vi "Test Window Frame Encode.vi"   [LabVIEW 2020]
doc: "Caraya unit test of RemoteVI Window Frame Encode.vi against tests/vectors (frame.json windowFrames), generated by tests/caraya/build.py - do not edit. One Assert Equal per vector, labelled with the vector's name; expected and actual are rendered as text by support/RemoteVI Check Window Frame Encode.vi (bytes as lowercase hex), so a failure shows both in the vector's own notation."
uses:
  <vilib>/addons/_JKI Toolkits/Caraya/classes/Test/Test.lvclass
  <vilib>/addons/_JKI Toolkits/Caraya/classes/Assert/Assert.lvclass
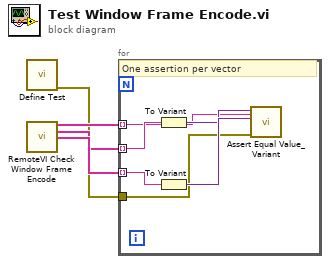
[diagram p0: block diagram]
diagram:
  n1 = call <vilib>:"Define Test.vi"() -> ("error out"=w1:errorcluster)  [unwired: 10 in, 1 out]
  n2 = call "RemoteVI Check Window Frame Encode.vi"() -> ("labels"=w2:string[], "expected"=w3:string[], "actual"=w4:string[])  [unwired: 12 in, 1 out]
  n3 = for {
    tunnel: w2 -> [w5] mode=indexing
    tunnel: w3 -> [w6] mode=indexing
    tunnel: w4 -> [w7] mode=indexing
    tunnel: w1 -> [w8]
    # "One assertion per vector"
    n4 = To Variant(anything=w6) -> (Variant=w9:variant)
    n5 = To Variant(anything=w7) -> (Variant=w10:variant)
    n6 = call <vilib>:"Assert Equal Value_Variant.vi"("Label"=w5, "error in (no error)"=w8, "Actual"=w10, "Expected"=w9) -> ()  [unwired: 6 in, 2 out]
  }
